vi "Fire User Event - Stop.vi"(8 "error in (no error)":errorcluster, 11 "User Events":T1) -> (0 "error out":errorcluster)   [LabVIEW 2020, in "User Event - Stop.lvlib"]
doc: "Send the Stop event to stop the Event Handling Loop."
uses:
  User Event - Stop.lvlib
  User Events.ctl
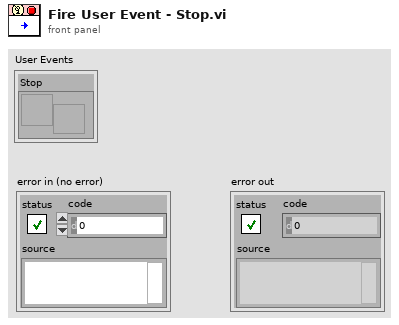
[diagram p1: front panel]
types:
  T1 = typedef "User Event - Stop.lvlib/User Events.ctl" = cluster{"Stop":refnum<user-event>}
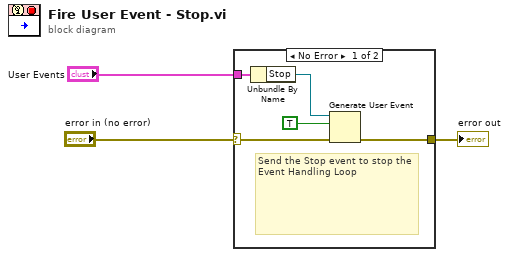
[diagram p0: block diagram]
diagram:
  n1 = case shown="No Error" "error in (no error)" {
    selector: "error in (no error)" -> [w6 w9]
    tunnel: [w7 w9] -> w3
    tunnel: "User Events" -> [w5 _]
    frame No Error {
      # "Send the Stop event to stop the Event Handling Loop"
      n2 = Unbundle By Name(w5) -> ("Stop"=w4:refnum<user-event>)
      n3 = Generate User Event(user event=w4, event data cluster=TRUE ("event data"), error in=w6) -> (error out=w7:errorcluster)  [unwired: 1 in, 1 out]
    }
    frame Error {
    }
  }
  "error out" <- w3
